vi "LTE check RB Offset.vi"(8 "error in (no error)":errorcluster caption="에러 입력(에러 없음)", 10 "RB Offset":i32, 11 "Instrument Manager 입력":refnum<class "Instrument Manager.lvclass">) -> (0 "error out":errorcluster caption="에러 출력", 2 "불리언":bool, 3 "Instrument Manager 출력":refnum<class "Instrument Manager.lvclass">)   [LabVIEW 2023, in "Instrument Manager.lvclass"]
uses:
  Instrument Manager.lvclass
  Instrument Manager.lvclass/Instrument Manager.ctl
  Module/ANRITSU Call Box/Type Definition/LTE RB Setting Params for query.ctl
  Module/ANRITSU Call Box/ANRITSU Call Box.lvlib
  Module/ANRITSU Call Box/Interface Class/Anritsu Call Box.lvclass
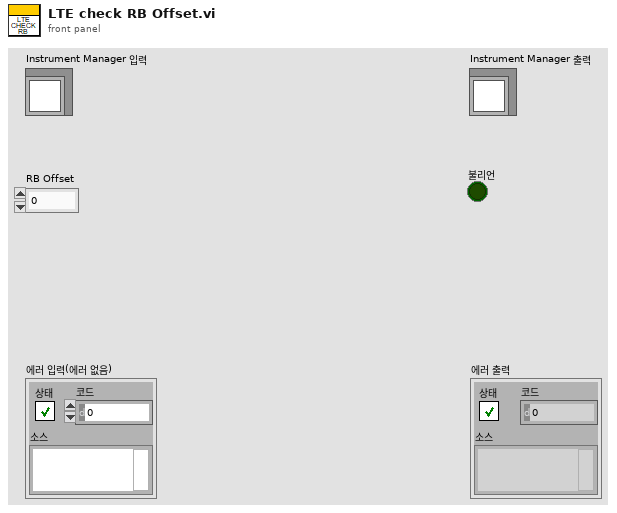
[diagram p1: front panel]
types:
  T1 = typedef "ANRITSU Call Box.lvlib/LTE RB Setting Params for query.ctl" = cluster{"Target CA Type":enum16{"PCC", "SCC1"}, "RB Setting Type":enum16{"Number of RB", "Starting RB"}}
  T2 = cluster{"Anritsu Call Box":refnum<class "Anritsu Call Box.lvclass">, "Spectrum Analyzer":refnum<class "Interface_Spectrum.lvclass">, "RF Switch Box":refnum<class "RF Filter Box.lvclass">, "Turn Table":refnum<class "Interface - Turn Table.lvclass">, "Mast":refnum<class "Interface - Mast.lvclass">, "3D Controller":refnum<class "Interface_3D Controller.lvclass">}
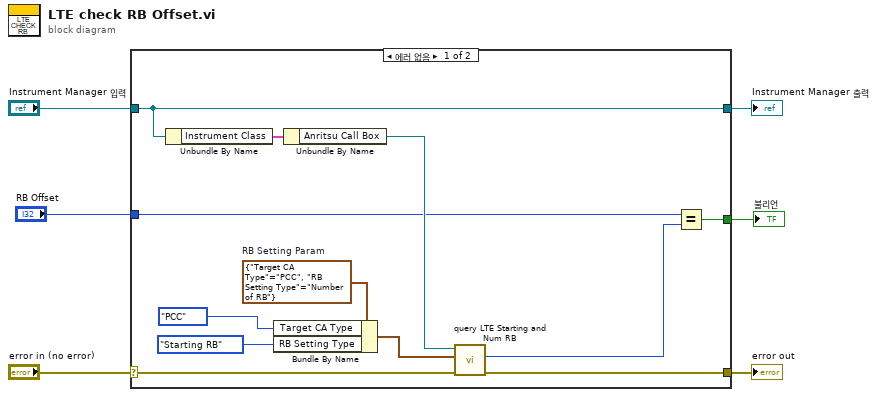
[diagram p0: block diagram]
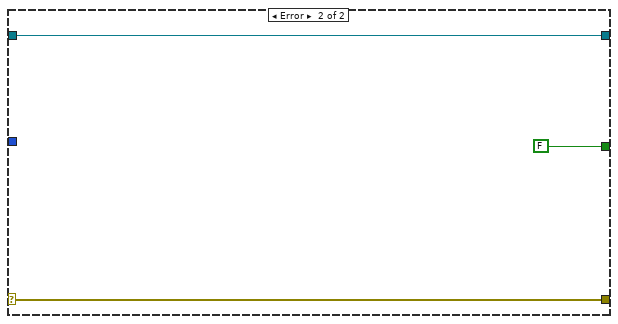
[diagram p2: hidden frame]
diagram:
  n1 = case shown="에러 없음" "error in (no error)" {
    selector: "error in (no error)" -> [w18 w21]
    tunnel: [w17 w21] -> w5
    tunnel: [w16 w20] -> w3
    tunnel: "Instrument Manager 입력" -> [w16 w20]
    tunnel: "RB Offset" -> [w8 _]
    tunnel: [w7 FALSE] -> w1
    frame No Error {
      w13 = T1 {"Target CA Type"=enum."PCC", "RB Setting Type"=enum."Number of RB"}  # RB Setting Param
      n2 = Unbundle By Name(w16) -> ("Instrument Class"=w15:T2)
      n3 = Bundle By Name(cluster=w13, "Target CA Type"=enum16{"PCC", "SCC1"}."PCC", "RB Setting Type"=enum16{"Number of RB", "Starting RB"}."Starting RB") -> (w12:T1)
      n4 = Unbundle By Name(w15) -> ("Anritsu Call Box"=w14:refnum<class "Anritsu Call Box.lvclass">)
      n5 = call-dynamic "query LTE Starting and Num RB.vi"("error in (no error)"=w18, "RB Setting Param"=w12, "Anritsu Call Box in"=w14) -> ("error out"=w17:errorcluster, "RB Value"=w9:i32)  [unwired: 6 in, 1 out]
      n6 = Equal?(x=w8, y=w9) -> (x = y?=w7:bool)
    }
    frame Error {
    }
  }
  "error out" <- w5
  "Instrument Manager 출력" <- w3
  "불리언" <- w1
